vi "PicoScope6000aRunBlock.vi"(7 "Acquisition Settings":T1 {"postTriggerSamples" format="%_6p"; "preTriggerSamples" format="%_6p"}, 8 "error in (no error)":errorcluster, 11 "handle in":i16) -> (0 "error out":errorcluster, 3 "handle out":i16, 4 "timeIndisposedMs":dbl, 6 "Total Requested Samples":u64)   [LabVIEW 2009]
doc: "Calls ps6000aRunBlock"
uses:
  ps6000a.dll
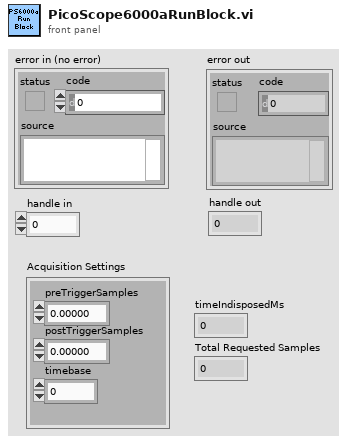
[diagram p1: front panel]
types:
  T1 = cluster{"preTriggerSamples":u64, "postTriggerSamples":u64, "timebase":u32}
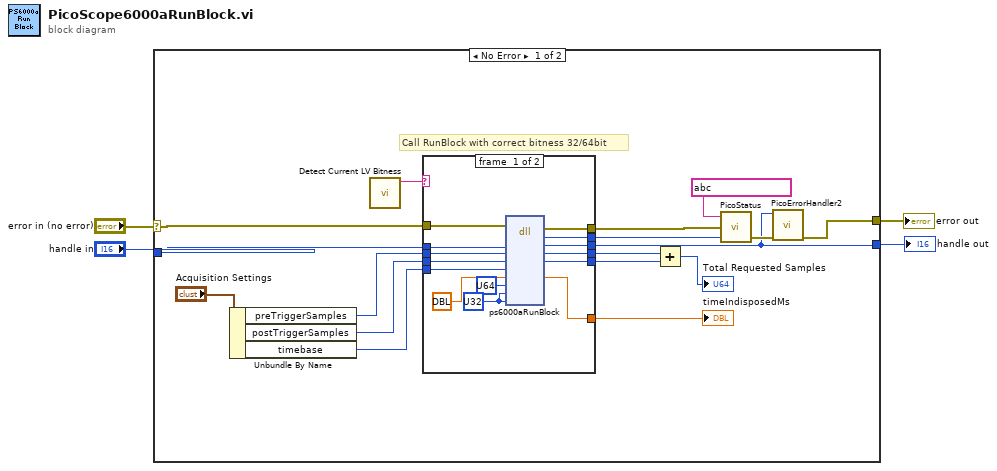
[diagram p0: block diagram]
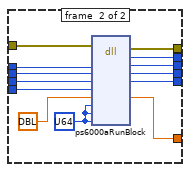
[diagram p2: hidden frame]
diagram:
  n1 = case shown="No Error" "error in (no error)" {
    selector: "error in (no error)" -> [w15 w50]
    tunnel: [w8 w50] -> w2
    tunnel: "handle in" -> [w14 w49]
    tunnel: [w7 w49] -> w3
    frame #0 {
      # "Call RunBlock with correct bitness 32/64bit"
      n2 = Unbundle By Name("Acquisition Settings") -> ("preTriggerSamples"=w13:u64, "postTriggerSamples"=w12:u64, "timebase"=w11:u32)
      n3 = call "Detect Current LV Bitness.vi"() -> ("bitness"=w9:string)  [unwired: 11 in]
      n4 = case shown="\"64\"" w9 {
        tunnel: [w35 w48] -> w21
        tunnel: [w34 w47] -> w20
        tunnel: [w33 w46] -> w18
        tunnel: [w32 w45] -> w17
        tunnel: w15 -> [w31 w44]
        tunnel: w14 -> [w30 w43]
        tunnel: w13 -> [w28 w41]
        tunnel: w12 -> [w27 w40]
        tunnel: w11 -> [w26 w39]
        tunnel: [w25 w38] -> w7
        tunnel: [w22 w36] -> w6
        frame #0 {
          w24 = u32 ? ("pParameter")
          n5 = dll-call lib="ps6000a.dll" fn="ps6000aRunBlock" ("ps3000.dll:_ps3000_open_unit@0")(error in=w31, "handle"=w30, "noOfPreTriggerSamples"=w28, "noOfPostTriggerSamples"=w27, "timebase"=w26, "timeIndisposedMs"=dbl ? ("pParameter"), "segmentIndex"=u64 ?, "lpReady"=w24, "pParameter"=w24) -> (error out=w32:errorcluster, "PICO_STATUS"=w33:u32, "handle"=w25:i16, "noOfPreTriggerSamples"=w35:u64, "noOfPostTriggerSamples"=w34:u64, "timeIndisposedMs"=w22:dbl)  [unwired: 6 in, 1 out]
        }
        frame #1 {
          w37 = u64 ? ("pParameter")
          n6 = dll-call lib="ps6000a.dll" fn="ps6000aRunBlock" ("ps3000.dll:_ps3000_open_unit@0")(error in=w44, "handle"=w43, "noOfPreTriggerSamples"=w41, "noOfPostTriggerSamples"=w40, "timebase"=w39, "timeIndisposedMs"=dbl ? ("pParameter"), "segmentIndex"=w37, "lpReady"=w37, "pParameter"=w37) -> (error out=w45:errorcluster, "PICO_STATUS"=w46:u32, "handle"=w38:i16, "noOfPreTriggerSamples"=w48:u64, "noOfPostTriggerSamples"=w47:u64, "timeIndisposedMs"=w36:dbl)  [unwired: 6 in, 1 out]
        }
      }
      "timeIndisposedMs" <- w6
      n7 = Add(x=w21, y=w20) -> (x+y=→"Total Requested Samples":u64)
      n8 = call "PicoStatus.vi"("PICO STATUS"=w18, "error in"=w17, "source"=string ?) -> ("error out"=w10:errorcluster)
      n9 = call "PicoErrorHandler2.vi"("error in (no error)"=w10, "handle In"=w7) -> ("error out"=w8:errorcluster)  [unwired: 9 in]
    }
    frame #1 {
    }
  }
  "error out" <- w2
  "handle out" <- w3
